vi "generate default line.vi"(7 "EthernetIP configuration":refnum<class "EIP Tags Configuration.lvclass">, 8 "error in":errorcluster, 11 "operations table":refnum<vi>) -> (0 "error out":errorcluster, 2 "line":T1)   [LabVIEW 2013, in "EIP Tags editor node.lvclass"]
uses:
  EIP Tags editor node.lvclass
  table line.ctl
  channel/EIP Tags Channel.lvclass
  configuration/EIP Tags Configuration.lvclass
  configuration/EIP Tags Configuration.lvclass/EIP Tags Configuration.ctl
  configuration/Read EIP tags.vi
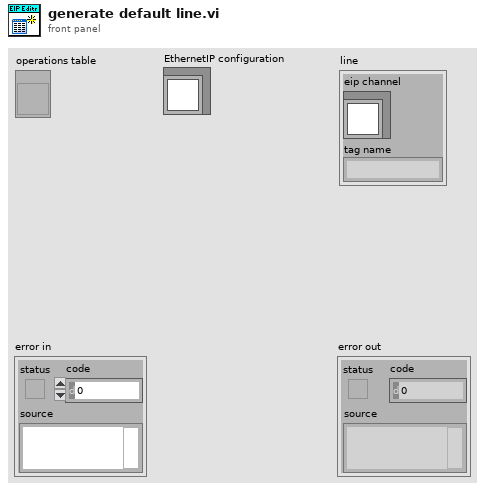
[diagram p1: front panel]
types:
  T1 = typedef "EIP Tags editor node.lvclass/table line.ctl" = cluster{"eip channel":refnum<class "EIP Tags Channel.lvclass">, "tag name":string}
  T2 = typedef "EIP Tags Configuration.lvclass/eip tag definition.ctl" = cluster{"eip tag types":T3, "unique tag name":string, "Number of Elements":u32}
  T3 = typedef "EIP Tags Configuration.lvclass/eip tag types.ctl" = enum16{"SINT", "INT", "DINT", "REAL", "BOOL", "STRING"}
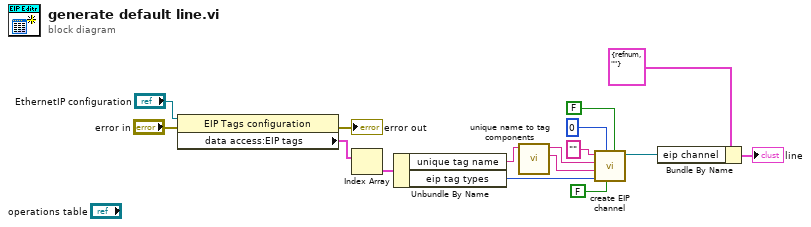
[diagram p0: block diagram]
diagram:
  n1 = property class="EIP Tags configuration"(reference="EthernetIP configuration", error in="error in") -> (error out=→"error out":errorcluster, "data access:EIP tags"=w8:T2[])  [unwired: 1 out]
  n2 = Index Array(array=w8) -> (element=w7:T2)  [unwired: 1 in]
  n3 = Unbundle By Name(w7) -> ("unique tag name"=w5:string, "eip tag types"=w2:T3)
  n4 = call "unique name to tag components.vi"("unique name"=w5) -> ("Tag Name"=w3:string, "Network Path"=w4:string)  [unwired: 9 in]
  n5 = call "create EIP channel.vi"("output?"=FALSE, "array?"=FALSE, "element index"=0, "eip tag type"=w2, "Tag Name"=w3, "Network Path"=w4, "name"="") -> ("EthernetIP Channel out"=w11:refnum<class "EIP Tags Channel.lvclass">)  [unwired: 4 in]
  n6 = Bundle By Name(cluster=T1 {"eip channel"=refnum, "tag name"=""} ("line"), "eip channel"=w11) -> (→"line":T1)
